vi "Test Process Trigger Broadcast.vi"(8 "error in (no error)":errorcluster, 11 "Process Test In":refnum<class "Process Test.lvclass">) -> (0 "error out":errorcluster, 3 "Process Test Out":refnum<class "Process Test.lvclass">)   [LabVIEW 2020, in "Process Test.lvclass"]
uses:
  Process Test.lvclass
  C:/Program Files (x86)/National Instruments/LabVIEW 2020/vi.lib/Astemes/LUnit/Test Case.lvclass
  Framework/Process/Process.lvclass/Process.ctl
  <vilib>/Astemes/LUnit/Test Case.lvclass/Test Case.ctl
  Framework/Process/Public/Lifecycle/Get Lifecycle State.vi
  Framework/Process/Protected/Messaging/Send Message.vi
  Framework/Broadcast Event Helpers/Execution timer.vi
  <vilib>/Astemes/LUnit/Set Assertion Type.vi
  <vilib>/Astemes/LUnit/Palette/Pass.vi
  <vilib>/Astemes/LUnit/Palette/Fail.vi
  Framework/Process/Private/SubVIs/Wait for finish.vi
  Framework/Process/Private/SubVIs/Set Lifecycle State.vi
  <vilib>/Utility/error.llb/Clear Errors.vi
  Framework/Process/Private/SubVIs/Handle Debug Data.vi
  <vilib>/Astemes/LUnit/Add test result.vi
  Framework/Logging/Log Debug.vi
  <vilib>/AdvancedString/1D String Array to Delimited String.vi
  <vilib>/Utility/High Resolution Relative Seconds.vi
  <vilib>/Astemes/LUnit/LUnit Record Assertion Result.vi
  <vilib>/Astemes/LUnit/LUnit Aggregate Assertion Results.vi
  <vilib>/Astemes/LUnit/Method Result/LUnit Merge Status.vi
  <vilib>/Astemes/LUnit/LUnit Concatenate result strings.vi
  <vilib>/Utility/error.llb/Error Cluster From Error Code.vi
  Framework/Process/Public/Read Name.vi
  Framework/Broadcast Event Helpers/Dequeue Broadcast Message.vi
  Framework/Process/Process.lvclass
  Process Test.lvclass/Process Test.ctl
  Framework/Broadcast Event Helpers/Broadcast Event Helpers.lvlib
  <vilib>/Astemes/LUnit/Test Case.lvclass
  C:/Git/astemes-triarc-framework/source/Framework Test Suite/Base Class Test/Base Test.lvclass
  C:/Git/astemes-triarc-framework/source/Framework Test Suite/Process Test/Process Test.lvclass
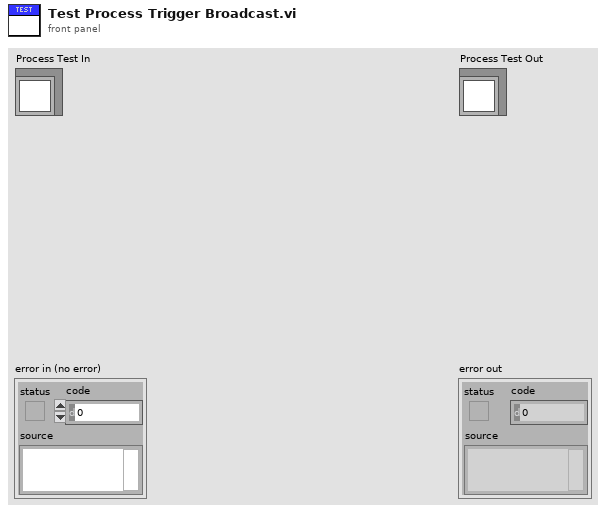
[diagram p1: front panel]
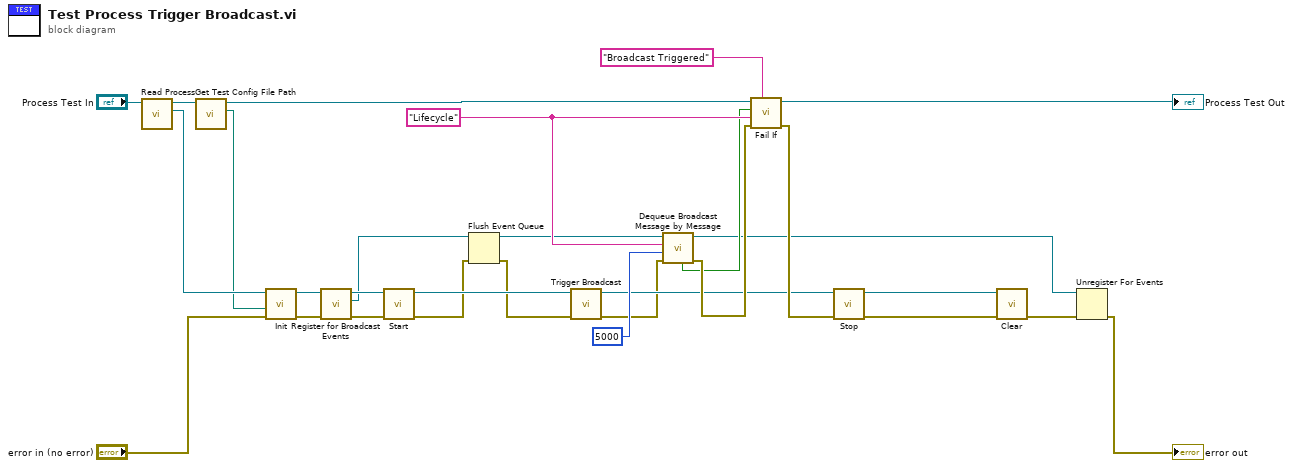
[diagram p0: block diagram]
diagram:
  w15 = "Lifecycle" ("Message")
  n1 = call "Read Process.vi"("Process Test in"="Process Test In") -> ("Process.lvclass"=w3:refnum<class "Process.lvclass">, "Process Test out"=w10:refnum<class "Process Test.lvclass">)  [unwired: 8 in, 1 out]
  n2 = call "Get Test Config File Path.vi"("Process Test In"=w10) -> ("Test config path"=w1:path, "Process Test Out"=w2:refnum<class "Process Test.lvclass">)  [unwired: 8 in, 1 out]
  n3 = call-dynamic "Init.vi"("error in (no error)"="error in (no error)", "Config File Path"=w1, "Process In"=w3) -> ("error out"=w28:errorcluster, "Process Out"=w29:refnum<class "Process.lvclass">)  [unwired: 7 in]
  n4 = call "Register for Broadcast Events.vi"("error in (no error)"=w28, "Process In"=w29) -> ("error out"=w22:errorcluster, "Event Registration Refnum Out"=w9:refnum<event-registration>, "Process Out"=w23:refnum<class "Process.lvclass">)  [unwired: 7 in]
  n5 = call "Start.vi"("error in (no error)"=w22, "Process In"=w23) -> ("error out"=w7:errorcluster, "Process Out"=w21:refnum<class "Process.lvclass">)  [unwired: 7 in, 1 out]
  n6 = Flush Event Queue(0:w9, 3:w7) -> (8:w8:refnum<event-registration>, 11:w5:errorcluster)  [unwired: 4 in, 1 out]
  n7 = call "Trigger Broadcast.vi"("error in (no error)"=w5, "Process in"=w21) -> ("error out"=w4:errorcluster, "Process out"=w6:refnum<class "Process.lvclass">)  [unwired: 8 in]
  n8 = call "Dequeue Broadcast Message by Message.vi"("error in (no error)"=w4, "Timeout (-1)"=5000, "Message"=w15, "Event Registration Refnum"=w8) -> ("error out"=w16:errorcluster, "Event Registration Refnum Out"=w12:refnum<event-registration>, "Timed Out?"=w14:bool)  [unwired: 3 in, 2 out]
  n9 = call <vilib>:"Fail If.vi"("Description"="Broadcast Triggered", "error in (no error)"=w16, "Message"=w15, "Fail?"=w14, "LUnit Test Case In"=w2) -> ("error out"=w17:errorcluster, "LUnit Test Case Out"=→"Process Test Out":refnum<class "Process Test.lvclass">)  [unwired: 5 in]
  n10 = call "Stop.vi"("error in (no error)"=w17, "Process In"=w6) -> ("error out"=w19:errorcluster, "Process Out"=w27:refnum<class "Process.lvclass">)  [unwired: 7 in, 1 out]
  n11 = call-dynamic "Clear.vi"("error in (no error)"=w19, "Process In"=w27) -> ("error out"=w26:errorcluster)  [unwired: 9 in]
  n12 = Unregister For Events(event registration refnum=w12, error in=w26) -> (error out=→"error out":errorcluster)
